vi "Init.vi"(8 "error in (no error)":errorcluster, 11 "Data in":refnum<class "CTI_GPIO_DigitalOut.lvclass">) -> (0 "error out":errorcluster, 3 "Data out":refnum<class "CTI_GPIO_DigitalOut.lvclass">)   [LabVIEW 2021, in "CTI_GPIO_DigitalOut.lvclass"]
doc: "Abstract Data Classes 2.1.1.13\nTim Streeter - TSA\nCopyright (c) 2025, TSA"
uses:
  CTI_GPIO_DigitalOut.lvclass
  <vilib>/CTI/CTI Drivers/CTI/GPIO Direction.ctl
  CTI_GPIO_DigitalOut.lvclass/CTI_GPIO_DigitalOut.ctl
  <vilib>/CTI/CTI Drivers/CTI/Session/Session.lvclass
  <vilib>/CTI/CTI Drivers/CTI/CTI.lvlib
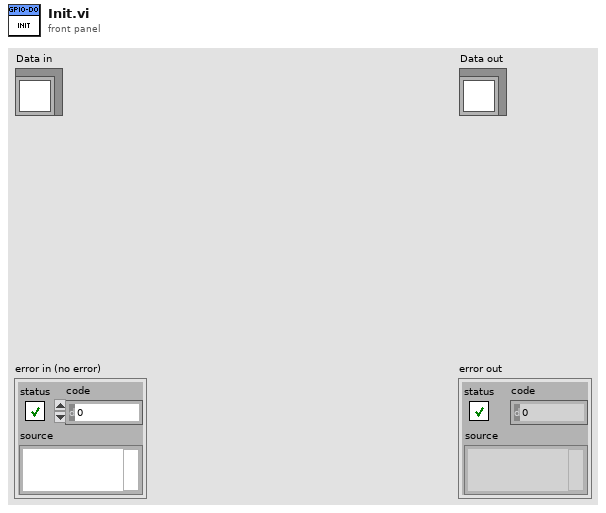
[diagram p1: front panel]
types:
  T1 = typedef "CTI.lvlib/GPIO Direction.ctl" = enum16{"In", "Out"}
  T2 = typedef "CTI.lvlib/GPIO Number.ctl" = i8
  T3 = typedef "CTI.lvlib/GPIO Pull.ctl" = enum16{"None", "Up", "Down", "Both"}
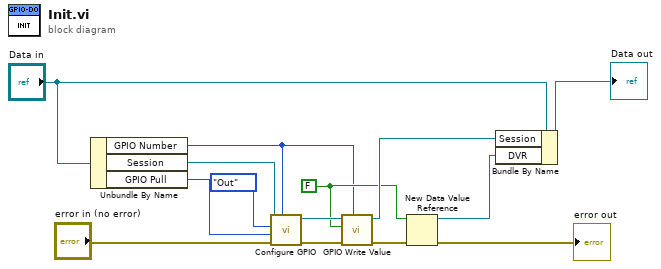
[diagram p0: block diagram]
diagram:
  w5 = FALSE
  n1 = Unbundle By Name("Data in") -> ("GPIO Number"=w1:T2, "Session"=w13:refnum<class "Session.lvclass">, "GPIO Pull"=w9:T3)
  n2 = call <vilib>:"Configure GPIO.vi"("GPIO #"=w1, "error in (no error)"="error in (no error)", "GPIO Pull (None)"=w9, "GPIO Direction"=GPIO_Direction."Out", "Session in"=w13) -> ("error out"=w8:errorcluster, "Session out"=w7:refnum<class "Session.lvclass">)  [unwired: 5 in]
  n3 = call <vilib>:"GPIO Write Value.vi"("GPIO #"=w1, "error in (no error)"=w8, "Value"=w5, "Session in"=w7) -> ("error out"=w4:errorcluster, "Session out"=w6:refnum<class "Session.lvclass">)  [unwired: 6 in]
  n4 = New Data Value Reference(data value=w5, error in=w4) -> (data value reference=w3:refnum<data-value>, error out=→"error out":errorcluster)
  n5 = Bundle By Name(cluster="Data in", "Session"=w6, "DVR"=w3) -> (→"Data out":refnum<class "CTI_GPIO_DigitalOut.lvclass">)
